vi "test_BuildBinaries.vi"() -> (3 "Pass?":bool)   [LabVIEW 2019, in "Tests.General.lvlib"]
uses:
  Tests.General.lvlib
  <vilib>/AppBuilder/AB_API_Simple/Build (path).vi
  <vilib>/regexp/Match Regular Expression.xnode
  <vilib>/AppBuilder/AB_API_Simple/NI_App_Builder_API.lvlib
panel:
  out "error out":errorcluster
  out "Generated files":path[](array[path])
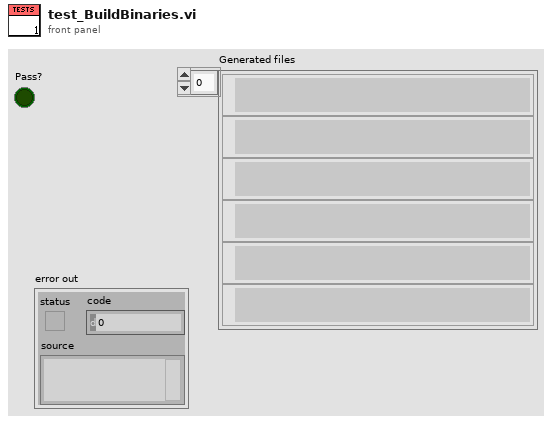
[diagram p1: front panel]
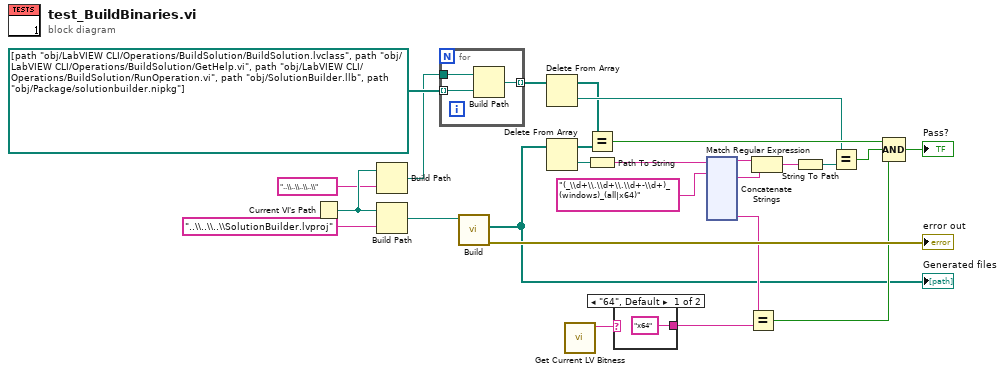
[diagram p0: block diagram]
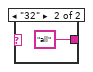
[diagram p2: hidden frame]
diagram:
  n1 = Current VI's Path() -> (path=w23:path)
  n2 = Build Path(base path=w23, name or relative path="..\\..\\..\\..\\") -> (appended path=w20:path)
  n3 = Build Path(base path=w23, name or relative path="..\\..\\..\\SolutionBuilder.lvproj") -> (appended path=w25:path)
  n4 = for {
    tunnel: path[] [path "obj/LabVIEW CLI/Operations/BuildSolution/BuildSolution.lvclass", path "obj/LabVIEW CLI/Operations/BuildSolution/GetHelp.vi", path "obj/LabVIEW CLI/Operations/BuildSolution/RunOperation.vi", path "obj/SolutionBuilder.llb", path "obj/Package/solutionbuilder.nipkg"] ("Generated files 2") -> [w28] mode=indexing
    tunnel: w20 -> [w29]
    tunnel: [w27] -> w6 mode=indexing
    n5 = Build Path(base path=w29, name or relative path=w28) -> (appended path=w27:path)
  }
  n6 = call-poly <vilib>:"Build.vi"("Path to project"=w25) -> ("error out"=→"error out":errorcluster, "Generated files"=w5:path[])  [unwired: 9 in]
  "Generated files" <- w5
  n7 = Delete From Array(array=w6) -> (deleted portion=w4:path, array with subset deleted=w3:path[])  [unwired: 2 in]
  n8 = Delete From Array(array=w5) -> (deleted portion=w1:path, array with subset deleted=w2:path[])  [unwired: 2 in]
  n9 = call <vilib>:"Get Current LV Bitness.vi"() -> ("bitness"=w10:string)  [unwired: 11 in]
  n10 = Equal?(x=w3, y=w2) -> (x = y?=w13:bool)
  n11 = Path To String(path=w1) -> (string=w18:string)
  n12 = case shown="\"64\", Default" w10 {
    tunnel: ["x64" ("name or relative path") "all" ("name or relative path")] -> w8
    frame "64", Default {
    }
    frame "32" {
    }
  }
  n13 = xnode "Match Regular Expression"("input string"=w18, "regular expression"="(_\\d+\\.\\d+\\.\\d+-\\d+)_(windows)_(all|x64)") -> ("before match"=w17:string, "after match"=w16:string, "submatch 3"=w9:string)  [unwired: 4 in, 5 out]
  n14 = Equal?(x=w9, y=w8) -> (x = y?=w7:bool)
  n15 = Concatenate Strings(w17, w16) -> (w15:string)
  n16 = String To Path(string=w15) -> (path=w14:path)
  n17 = Equal?(x=w4, y=w14) -> (x = y?=w12:bool)
  n18 = Compound Arithmetic op=AND(w13, w12, w7) -> (→"Pass?":bool)
